vi "Example.vi"() -> ()   [LabVIEW 2021]
uses:
  Children/Serial/CTI_Serial_Bus.lvclass
  C:/Program Files (x86)/National Instruments/LabVIEW 2021/vi.lib/TSA/Omni-Bus/Omni-Bus/Bus Access/Bus_Access.lvclass
  Channels/GPIO/DigitalOut/CTI_GPIO_DigitalOut.lvclass
  C:/Program Files (x86)/National Instruments/LabVIEW 2021/vi.lib/TSA/Abstract Data Classes/Abs_Types/Value/Abs_Value.lvclass
  <vilib>/TSA/Omni-Bus/Omni-Bus/Omni_Bus.lvclass
  <vilib>/CTI/CTI Drivers/CTI/GPIO Number.ctl
  <vilib>/CTI/CTI Drivers/CTI/GPIO Pull.ctl
  Channels/Analog In/CTI_AnalogIn.lvclass
  <vilib>/CTI/CTI Drivers/CTI/ADC Number.ctl
  <vilib>/TSA/Omni-Bus/Omni-Bus/Support/Read/Read U16.vi
  <vilib>/TSA/Omni-Bus/Omni-Bus/Support/Write/Write Boolean.vi
  <vilib>/TSA/Abstract Data Classes/Abs_Types/U16 Integer/Abs_U16 Integer.lvclass
  C:/Program Files (x86)/National Instruments/LabVIEW 2021/vi.lib/TSA/Abstract Data Classes/Abs_Types/Type/Abs_Type.lvclass
  <vilib>/TSA/Abstract Data Classes/Abs_Types/Boolean/Abs_Boolean.lvclass
  <vilib>/TSA/Omni-Bus/Omni-Bus/Support/FindVar.vi
  <vilib>/CTI/CTI Drivers/CTI/CTI.lvlib
panel:
  out "Numeric":u16
  out "Analog In":dbl
  out "error out 2":errorcluster
  out "error out":errorcluster
  in  "Digital Out":bool
  in  "stop":bool
  out "Tags":string[](array[string])
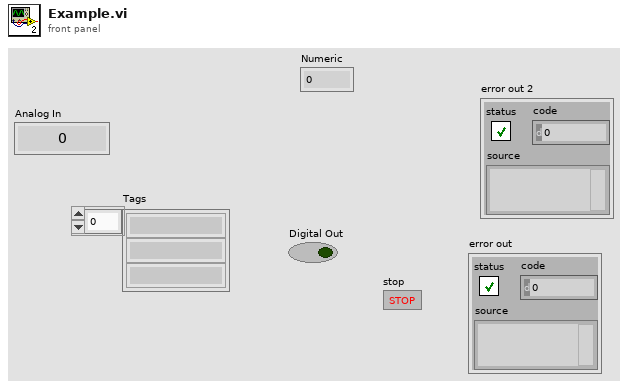
[diagram p1: front panel]
types:
  T1 = typedef "CTI.lvlib/ADC Number.ctl" = i8
  T2 = typedef "CTI.lvlib/GPIO Pull.ctl" = enum16{"None", "Up", "Down", "Both"}
  T3 = typedef "CTI.lvlib/GPIO Number.ctl" = i8
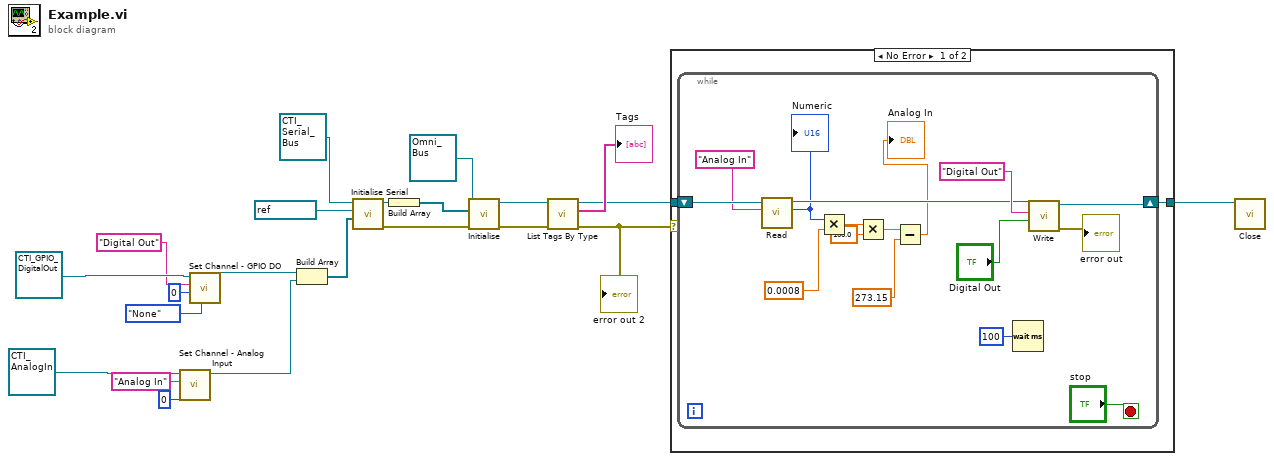
[diagram p0: block diagram]
diagram:
  n1 = call "Set Channel - Analog Input.vi"("ADC Number"=T1 0, "Tag"="Analog In", "CTI_GPIO_DigitalOut in"=refnum<class "CTI_AnalogIn.lvclass"> refnum) -> ("CTI_GPIO_DigitalOut out"=w5:refnum<class "CTI_AnalogIn.lvclass">)  [unwired: 7 in, 1 out]
  n2 = call "Set Channel - GPIO DO.vi"("GPIO Pull"=GPIO_Pull."None", "GPIO Number"=T3 0, "Tag"="Digital Out", "CTI_GPIO_DigitalOut in"=refnum<class "CTI_GPIO_DigitalOut.lvclass"> refnum ("CTI_GPIO_DigitalOut.lvclass")) -> ("CTI_GPIO_DigitalOut out"=w3:refnum<class "CTI_GPIO_DigitalOut.lvclass">)  [unwired: 6 in, 1 out]
  n3 = Build Array(w3, w5) -> (w20:refnum<class "Abs_Value.lvclass">[])
  n4 = call "Initialise Serial.vi"("Channels"=w20, "VISA resource name"=refnum<visa-resource-name> "COM3", "CTI_Serial_Bus in"=refnum<class "CTI_Serial_Bus.lvclass"> refnum) -> ("error out"=w10:errorcluster, "CTI_Serial_Bus out"=w18:refnum<class "CTI_Serial_Bus.lvclass">)  [unwired: 7 in]
  n5 = Build Array(w18) -> (w19:refnum<class "CTI_Serial_Bus.lvclass">[])
  n6 = call-dynamic "Initialise.vi"("error in (no error)"=w10, "Bus Access"=w19, "Var Bus in"=refnum<class "Omni_Bus.lvclass"> refnum) -> ("error out"=w11:errorcluster, "Var Bus out"=w16:refnum<class "Omni_Bus.lvclass">)  [unwired: 7 in]
  n7 = call <vilib>:"List Tags By Type.vi"("error in (no error)"=w11, "Var Bus in"=w16) -> ("error out"=w12:errorcluster, "Tags"=→"Tags":string[], "Var Bus out"=w14:refnum<class "Omni_Bus.lvclass">)  [unwired: 6 in, 1 out]
  "error out 2" <- w12
  n8 = case shown="No Error" w12 {
    tunnel: w14 -> [w24 w41]
    tunnel: [w23 w41] -> w13
    frame No Error {
      n9 = while {
        shift-right: [w39] -> w23
        shift-left: w24 -> [w35]
        stop <- "stop" stop-if-true
        n10 = call-poly <vilib>:"Read.vi"("Tag"="Analog In", "Var Bus in"=w35) -> ("Numeric"=w31:u16, "Var Bus out"=w34:refnum<class "Omni_Bus.lvclass">)  [unwired: 7 in, 1 out]
        "Numeric" <- w31
        n11 = Multiply(x=w31, y=0.0008) -> (x*y=w29:dbl)
        n12 = Multiply(x=w29, y=100.0) -> (x*y=w27:dbl)
        n13 = Subtract(x=w27, y=273.15) -> (x-y=→"Analog In":dbl)
        n14 = Wait (ms)(milliseconds to wait=u32 100) -> ()  [unwired: 1 out]
        n15 = call-poly <vilib>:"Write.vi"("Boolean"="Digital Out", "Tag"="Digital Out", "Omni_Bus in"=w34) -> ("error out"=→"error out":errorcluster, "Omni_Bus out"=w39:refnum<class "Omni_Bus.lvclass">)  [unwired: 7 in]
      }
    }
    frame Error {
    }
  }
  n16 = call-dynamic "Close.vi"("Data in"=w13) -> ()  [unwired: 9 in, 2 out]
